vi "Get Boolean Channel Name.vi"(9 "Channel Numer":i32, 11 "Input?":bool) -> (1 "Bool Channel Name":string, 2 "Bool Channel ID":string)   [LabVIEW 2026, in "Modbus.lvlib" / "Modbus.lvclass"]
uses:
  Modbus.lvclass
  Globals/Modbus Strings.vi
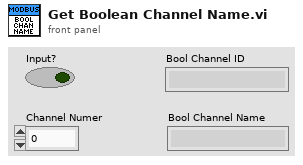
[diagram p1: front panel]
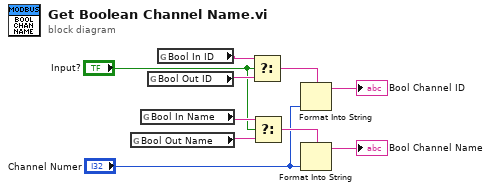
[diagram p0: block diagram]
diagram:
  n1 = global read "Modbus Strings.vi" "Bool Out Name"() -> (w5:string)
  n2 = global read "Modbus Strings.vi" "Bool In Name"() -> (w6:string)
  n3 = global read "Modbus Strings.vi" "Bool Out ID"() -> (w10:string)
  n4 = global read "Modbus Strings.vi" "Bool In ID"() -> (w9:string)
  n5 = Select(t=w9, s="Input?", f=w10) -> (s? t:f=w8:string)
  n6 = Select(t=w6, s="Input?", f=w5) -> (s? t:f=w3:string)
  n7 = Format Into String(format string=w8, "Channel Numer") -> (resulting string=→"Bool Channel ID":string)  [unwired: 2 in, 1 out]
  n8 = Format Into String(format string=w3, "Channel Numer") -> (resulting string=→"Bool Channel Name":string)  [unwired: 2 in, 1 out]
